vi "Handle Packet Validation Error.vi"(9 "Packet Validation Error":errorcluster, 10 "ControlPacket":refnum<class "ControlPacket.lvclass">, 11 "Session in":refnum<class "Session.lvclass">) -> (0 "error out":errorcluster, 3 "Session out":refnum<class "Session.lvclass">)   [LabVIEW 2013, in "MQTT Base.lvlib" / "Session.lvclass"]
uses:
  Session.lvclass
  <vilib>/LabVIEW Open Source Project/MQTT Control Packets/Control Packets/ControlPacket/ControlPacket.lvclass
  Session Disconnection Reason -- enum.ctl
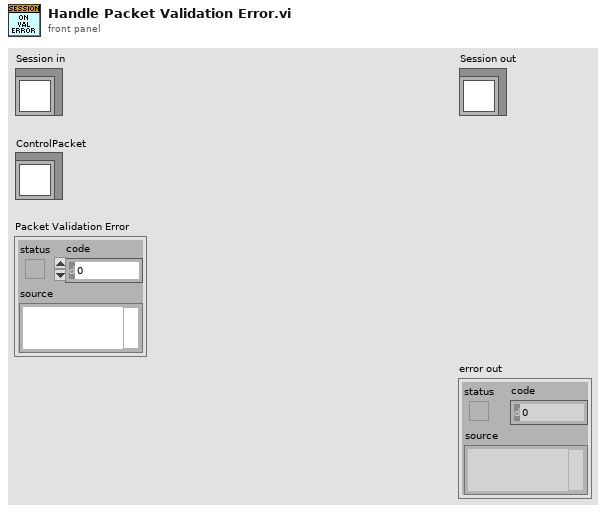
[diagram p1: front panel]
types:
  T1 = typedef "MQTT Base.lvlib/Session.lvclass/Session Disconnection Reason -- enum.ctl" = enum16{"Normal Stop", "Protocol Violation", "Disconnected by Peer"}
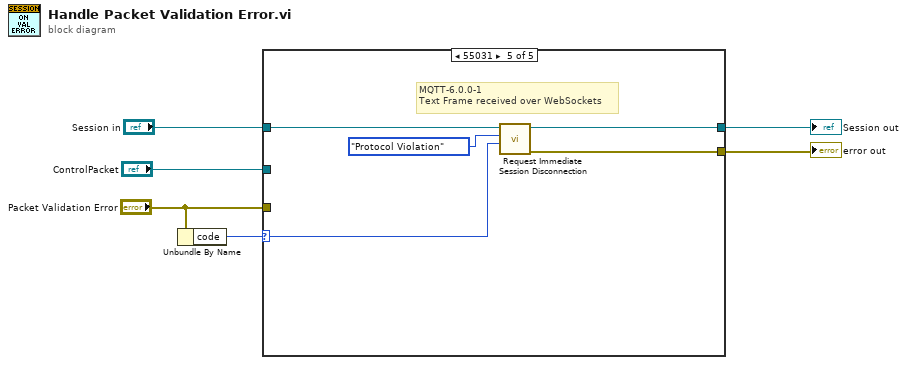
[diagram p0: block diagram]
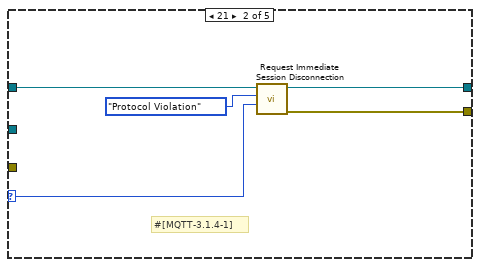
[diagram p3: hidden frame]
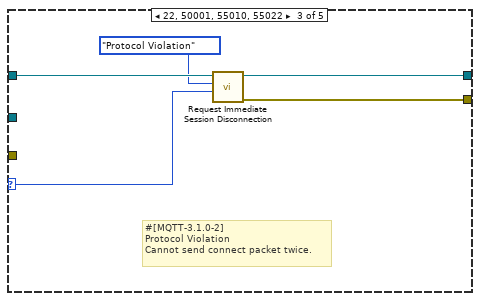
[diagram p4: hidden frame]
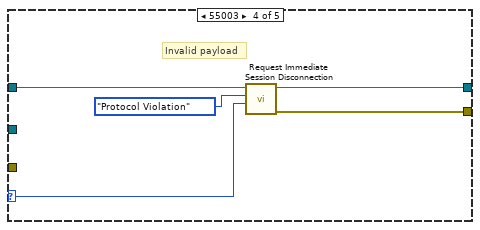
[diagram p5: hidden frame]
diagram:
  n1 = Unbundle By Name("Packet Validation Error") -> ("code"=w4:i32)
  n2 = case shown="55031" w4 {
    selector: w4 -> [_ w8 w13 w18 w23]
    tunnel: "Session in" -> [w7 w11 w17 w21 w26]
    tunnel: "ControlPacket" -> [_ _ _ _ _]
    tunnel: "Packet Validation Error" -> [_ _ _ _ _]
    tunnel: [w7 w10 w15 w20 w25] -> w2
    tunnel: [_ w9 w16 w19 w24] -> w1
    frame Default {
    }
    frame 21 {
      # "#[MQTT-3.1.4-1]"
      n3 = call "Request Immediate Session Disconnection.vi"("Protocol Violation Error Code"=w8, "Disconnection Reason"=Session_Disconnection_Reason_--_enum."Protocol Violation", "Session in"=w11) -> ("error out"=w9:errorcluster, "Session out"=w10:refnum<class "Session.lvclass">)  [unwired: 7 in]
    }
    frame 22, 50001, 55010, 55022 {
      # "#[MQTT-3.1.0-2]\nProtocol Violation\nCannot send connect packet twice."
      n4 = call "Request Immediate Session Disconnection.vi"("Protocol Violation Error Code"=w13, "Disconnection Reason"=Session_Disconnection_Reason_--_enum."Protocol Violation", "Session in"=w17) -> ("error out"=w16:errorcluster, "Session out"=w15:refnum<class "Session.lvclass">)  [unwired: 7 in]
    }
    frame 55003 {
      # "Invalid payload"
      n5 = call "Request Immediate Session Disconnection.vi"("Protocol Violation Error Code"=w18, "Disconnection Reason"=Session_Disconnection_Reason_--_enum."Protocol Violation", "Session in"=w21) -> ("error out"=w19:errorcluster, "Session out"=w20:refnum<class "Session.lvclass">)  [unwired: 7 in]
    }
    frame 55031 {
      # "MQTT-6.0.0-1\nText Frame received over WebSockets"
      n6 = call "Request Immediate Session Disconnection.vi"("Protocol Violation Error Code"=w23, "Disconnection Reason"=Session_Disconnection_Reason_--_enum."Protocol Violation", "Session in"=w26) -> ("error out"=w24:errorcluster, "Session out"=w25:refnum<class "Session.lvclass">)  [unwired: 7 in]
    }
  }
  "error out" <- w1
  "Session out" <- w2
